vi "SetTestv3NoRbac.vi"() -> ()   [LabVIEW 2017]
uses:
  <vilib>/httpClient/PUTBuffer.vi
  <vilib>/httpClient/LabVIEWHTTPClient.lvlib
  <vilib>/Analysis/NI_AALBase.lvlib
panel:
  out "body":string
  out "result string":string
  out "standard deviation":dbl format="%0.2f"
  out "mean":dbl format="%0.2f"
  out "error out":errorcluster
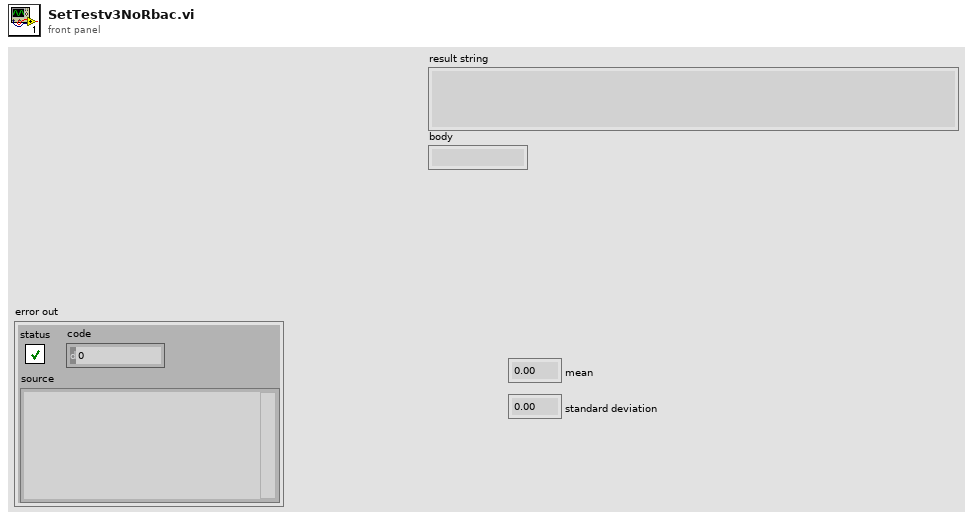
[diagram p1: front panel]
types:
  T1 = cluster{"dbl_field":dbl, "string_field":string, "long_field":i64, "int_array_field":i32[]}
  T2 = typedef "LabVIEWHTTPClient.lvlib/ClientHandle.ctl" = refnum<k1>
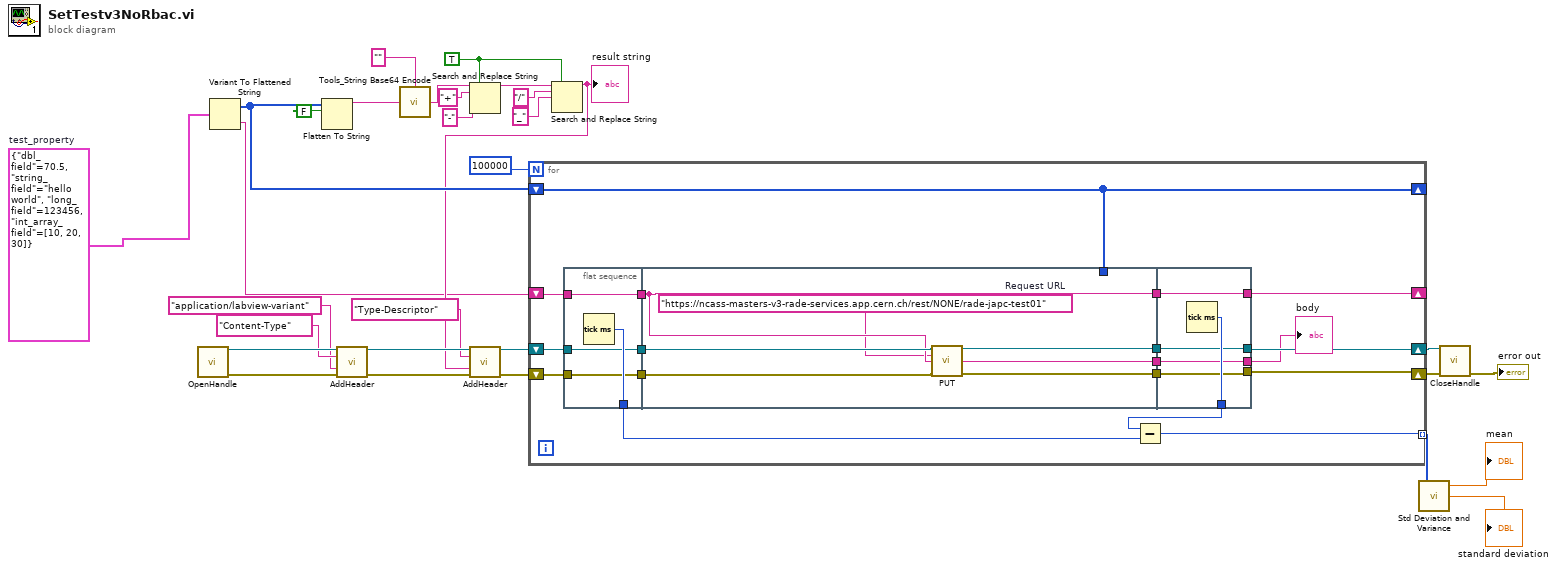
[diagram p0: block diagram]
diagram:
  w1 = T1 {"dbl_field"=70.5, "string_field"="hello world", "long_field"=123456, "int_array_field"=[10, 20, 30]}  # test_property
  w7 = TRUE ("replace all? (F)")
  n1 = call <vilib>:"OpenHandle.vi"() -> ("client handle out"=w26:T2, "error out"=w27:errorcluster)  [unwired: 14 in]
  n2 = Variant To Flattened String(Variant=w1) -> (data string=w2:string, 1:w19:i16[])
  n3 = Flatten To String(anything=w19, prepend array or string size? (T)=FALSE) -> (data string=w25:string)  [unwired: 2 in, 2 out]
  n4 = call <vilib>:"AddHeader.vi"("client handle"=w26, "header"="Content-Type", "value"="application/labview-variant", "error in (no error)"=w27) -> ("client handle out"=w28:T2, "error out"=w29:errorcluster)  [unwired: 10 in]
  n5 = call <userlib>:"Tools_String Base64 Encode.vi"("Normal String"=w25, "Line separator (\\n)"="") -> ("Base64 String"=w9:string)
  n6 = Search and Replace String(replace all?=w7, input string=w9, search string="+" ("substring (\"\")"), replace string="-" ("replace string (\"\")")) -> (result string=w8:string)  [unwired: 4 in, 3 out]
  n7 = Search and Replace String(replace all?=w7, input string=w8, search string="/" ("substring (\"\")"), replace string="_" ("replace string (\"\")")) -> (result string=w4:string)  [unwired: 4 in, 3 out]
  "result string" <- w4
  n8 = call <vilib>:"AddHeader.vi"("client handle"=w28, "header"="Type-Descriptor", "value"=w4, "error in (no error)"=w29) -> ("client handle out"=w12:T2, "error out"=w20:errorcluster)  [unwired: 10 in]
  n9 = for {
    N: 100000 -> [_]
    shift-right: [w48] -> _
    shift-left: w19 -> [w48]
    tunnel: [w45] -> w15 mode=indexing
    shift-right: [w39] -> w17
    shift-left: w12 -> [w43]
    shift-right: [w37] -> w16
    shift-left: w20 -> [w41]
    shift-right: [w32] -> _
    shift-left: w2 -> [w34]
    n10 = flat-sequence {
      tunnel: [w52] -> w47
      tunnel: [w51] -> w44
      tunnel: w43 -> [w51]
      tunnel: [w50] -> w42
      tunnel: w41 -> [w50]
      tunnel: [w49] -> w35
      tunnel: w34 -> [w49]
      tunnel: w48 -> [_]
      tunnel: w44 -> [w59]
      tunnel: w42 -> [w58]
      tunnel: [w57] -> w40
      tunnel: [w56] -> w38
      tunnel: [w55] -> w36
      tunnel: w35 -> [w54]
      tunnel: [w54] -> w33
      tunnel: [w64] -> w46
      tunnel: w40 -> [w63]
      tunnel: [w63] -> w39
      tunnel: [w62] -> w37
      tunnel: w38 -> [w62]
      tunnel: [w61] -> w31
      tunnel: w36 -> [w61]
      tunnel: w33 -> [w60]
      tunnel: [w60] -> w32
      frame #0 {
        n11 = Tick Count (ms)() -> (millisecond timer value=w52:u32)
      }
      frame #1 {
        w53 = "https://ncass-masters-v3-rade-services.app.cern.ch/rest/NONE/rade-japc-test01"  # Request URL
        n12 = call-poly <vilib>:"PUT.vi"("client handle"=w59, "url"=w53, "buffer"=w54, "error in (no error)"=w58) -> ("client handle out"=w57:T2, "body"=w55:string, "error out"=w56:errorcluster)  [unwired: 8 in, 1 out]
      }
      frame #2 {
        n13 = Tick Count (ms)() -> (millisecond timer value=w64:u32)
      }
    }
    n14 = Subtract(x=w46, y=w47) -> (x-y=w45:u32)
    "body" <- w31
  }
  n15 = call <vilib>:"Std Deviation and Variance.vi"("X"=w15) -> ("mean"=→"mean":dbl, "standard deviation"=→"standard deviation":dbl)  [unwired: 1 in, 1 out]
  n16 = call <vilib>:"CloseHandle.vi"("client handle"=w17, "error in (no error)"=w16) -> ("error out"=→"error out":errorcluster)  [unwired: 13 in]
